vi "gen scan waveforms v3.vi"(4 "Scanner calibration":cluster{"Offset":dbl, "Amplitude":dbl}[](array[cluster])=[{"Offset"=2.5, "Amplitude"=-0.20500000000000002}, {"Offset"=2.5, "Amplitude"=0.0}, {"Offset"=2.69, "Amplitude"=0.0}, {"Offset"=2.55, "Amplitude"=0.0}] {"Amplitude" min=-5.0 max=5.0 step=0.005; "Offset" min=0.0 max=5.0 step=0.005}, 6 "Signal delays":T2={"ETL delay (samples)"=10, "Scanner delay (samples)"=-25, "Laser delay (samples)"=262}, 7 "Z Slices":cluster{"start":dbl, "delta":dbl, "end":dbl}={"start"=0.0, "delta"=0.0, "end"=1.0}, 8 "AO sample rate":dbl=100000.0 format="%.2p", 9 "Flash duration (s)":dbl, 10 "frame period (s)":dbl=0.006, 11 "volume period (s)":dbl) -> (1 "Digital signals":u8[][](array[numeric]), 2 "Analog signals":dbl[][](array[numeric]))   [LabVIEW 2020, in "Scan Generators.lvlib"]
uses:
  Scan Generators.lvlib
  <vilib>/Analysis/baseanly.llb/Scale 1D.vi
  <vilib>/Analysis/1siggen.llb/Ramp Pattern by Delta.vi
  <vilib>/Waveform/DWDTOps.llb/DWDT Boolean Array to Digital.vi
  <vilib>/Analysis/NI_AALBase.lvlib
panel:
  out "Mixed Signal Graph":T1(graph)
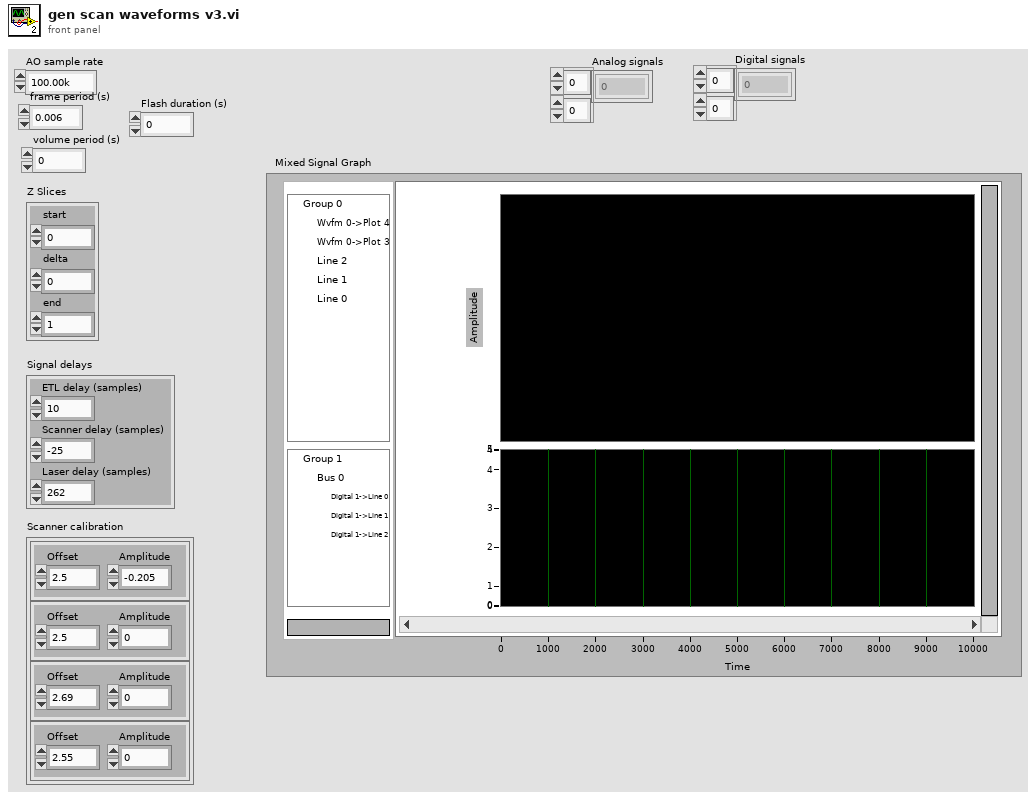
[diagram p1: front panel]
types:
  T1 = cluster{"Analog Waveforms 2":dbl[][], "digital waveform":digitalwaveform}
  T2 = cluster{"ETL delay (samples)":i32, "Scanner delay (samples)":i32, "Laser delay (samples)":i32}
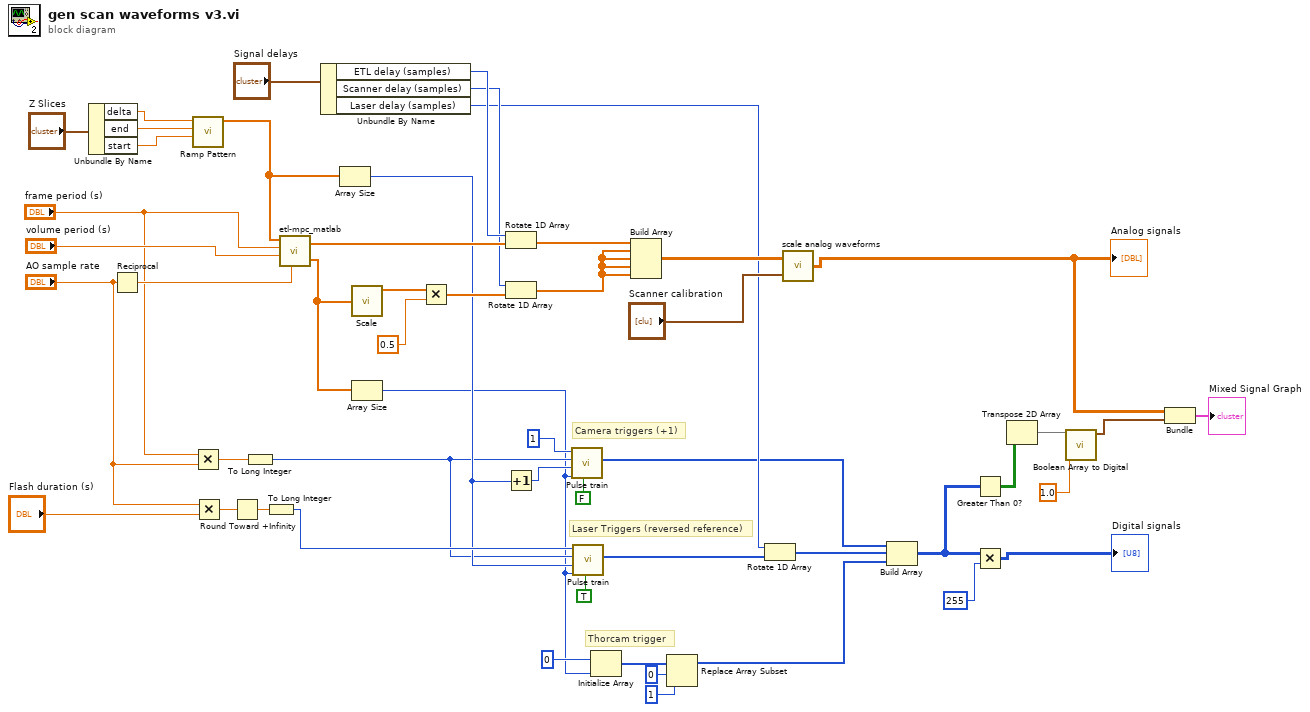
[diagram p0: block diagram]
diagram:
  # "Thorcam trigger"
  # "Laser Triggers (reversed reference)"
  # "Camera triggers (+1)"
  n1 = Unbundle By Name("Z Slices") -> ("delta"=w42:dbl, "end"=w43:dbl, "start"=w44:dbl)
  n2 = Reciprocal(x="AO sample rate") -> (1/x=w41:dbl)
  n3 = call-poly <vilib>:"Ramp Pattern.vi"("start"=w44, "end"=w43, "delta"=w42) -> ("Ramp Pattern"=w19:dbl[])  [unwired: 6 in, 2 out]
  n4 = Multiply(x="frame period (s)", y="AO sample rate") -> (x*y=w20:dbl)
  n5 = Multiply(x="AO sample rate", y="Flash duration (s)") -> (x*y=w25:dbl)
  n6 = Round Toward +Infinity(x=w25) -> (ceil(x): smallest int >= x=w24:dbl)
  n7 = To Long Integer(number=w20) -> (32bit integer=w15:i32)
  n8 = To Long Integer(number=w24) -> (32bit integer=w26:i32)
  n9 = call "etl-mpc_matlab.vi"("AO Sample Period"=w41, "volume period"="volume period (s)", "frame period"="frame period (s)", "slice array"=w19) -> ("Predicted Scan Path"=w18:dbl[], "ETL scan waveform"=w35:dbl[])  [unwired: 2 in]
  n10 = Unbundle By Name("Signal delays") -> ("ETL delay (samples)"=w34:i32, "Scanner delay (samples)"=w33:i32, "Laser delay (samples)"=w13:i32)
  n11 = Array Size(array=w19) -> (size(s)=w16:i32)
  n12 = call-poly <vilib>:"Scale.vi"("X"=w18) -> ("Y=(X-offset)/scale"=w39:dbl[])  [unwired: 3 out]
  n13 = Array Size(array=w18) -> (size(s)=w10:i32)
  n14 = Multiply(x=w39, y=0.5) -> (x*y=w36:dbl[])
  n15 = Rotate 1D Array(1:w35, 2:w34) -> (0:w32:dbl[])
  n16 = Rotate 1D Array(1:w36, 2:w33) -> (0:w31:dbl[])
  n17 = Increment(x=w16) -> (x+1=w17:i32)
  n18 = call "Pulse train.vi"("Reverse?"=FALSE, "Total length"=w10, "Cycles"=w17, "Cycle length"=w15, "Pulse length"=1) -> ("output array"=w5:u8[])  [unwired: 6 in]
  n19 = call "Pulse train.vi"("Reverse?"=TRUE, "Total length"=w10, "Cycles"=w16, "Cycle length"=w15, "Pulse length"=w26) -> ("output array"=w14:u8[])  [unwired: 6 in]
  n20 = Initialize Array(u8 0 ("element"), w10) -> (w9:u8[])
  n21 = Build Array(w32, w31, w31, w31, w31) -> (w30:dbl[][])
  n22 = Replace Array Subset(array=w9, new element=u8 1 ("new element/subarray"), index=0) -> (w4:u8[])
  n23 = Rotate 1D Array(1:w14, 2:w13) -> (0:w6:u8[])
  n24 = call "scale analog waveforms.vi"("Scaling parameters"="Scanner calibration", "Analog Waveforms"=w30) -> ("Analog Waveforms 2"=w47:dbl[][])
  "Analog signals" <- w47
  n25 = Build Array(w5, w6, w4) -> (w3:u8[][])
  n26 = Greater Than 0?(x=w3) -> (x > 0?=w50:bool[][])
  n27 = Multiply(x=w3, y=u8 255) -> (x*y=→"Digital signals":u8[][])
  n28 = Transpose 2D Array(2D array=w50) -> (transposed array=w49:bool[][])
  n29 = call-poly <vilib>:"Boolean Array to Digital.vi"("sample rate"=1.0, "boolean array"=w49) -> ("digital waveform"=w46:digitalwaveform)  [unwired: 8 in, 1 out]
  n30 = Bundle("Analog Waveforms 2"=w47, "digital waveform"=w46) -> (→"Mixed Signal Graph":T1)  [unwired: 1 in]
